vi "DeltaRAWdata(SubVI).vi"(1 "Value 3":u16[][](array[numeric]), 3 "error input":errorcluster) -> (5 "Robot-Delta 2":T1, 8 "error out":errorcluster)   [LabVIEW 2019]
panel:
  in  "Robot-Delta":T1
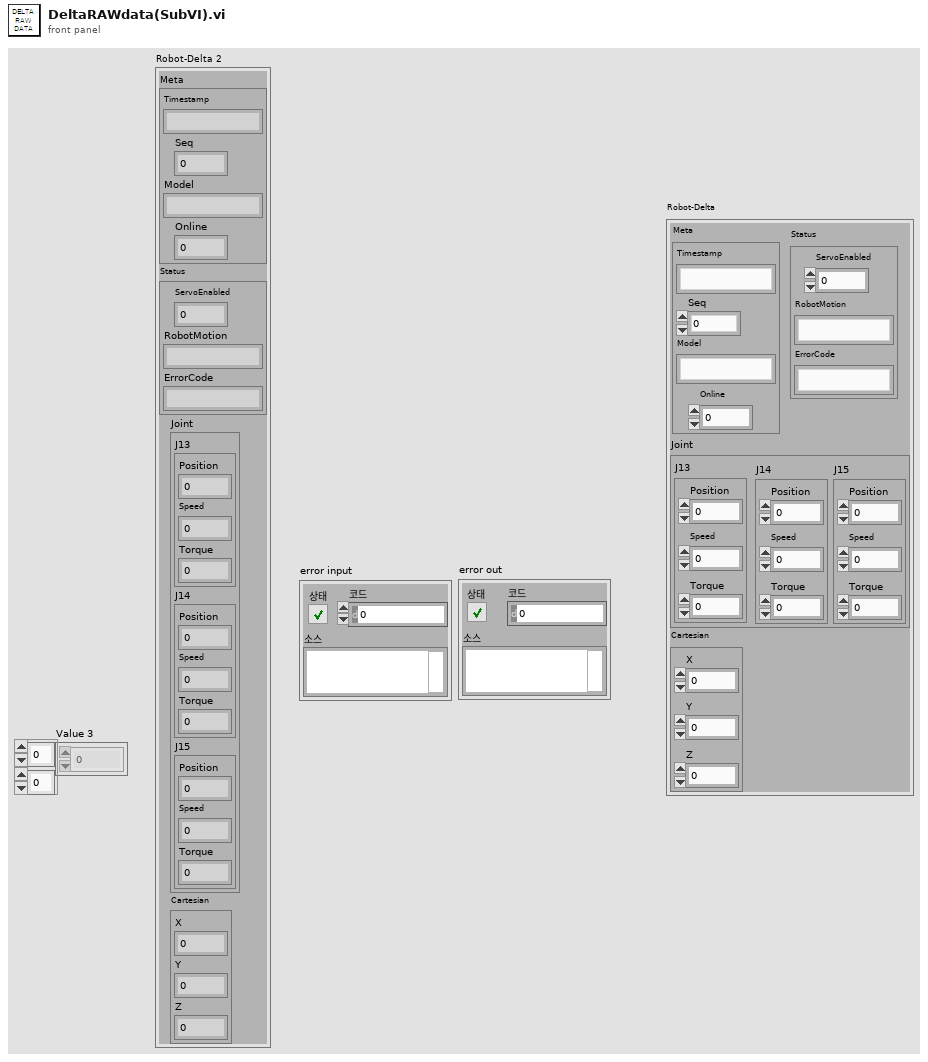
[diagram p1: front panel]
types:
  T1 = cluster{"Meta":cluster{"Timestamp":string, "Seq":dbl, "Model":string, "Online":dbl}, "Status":cluster{"ServoEnabled":dbl, "RobotMotion":string, "ErrorCode":string}, "Joint":cluster{"J13":cluster{"Position":dbl, "Speed":dbl, "Torque":dbl}, "J14":cluster{"Position":dbl, "Speed":dbl, "Torque":dbl}, "J15":cluster{"Position":dbl, "Speed":dbl, "Torque":dbl}}, "Cartesian":cluster{"X":dbl, "Y":dbl, "Z":dbl}}
  T2 = cluster{"[0]":u16, "[1]":u16, "[2]":u16, "[3]":u16, "[4]":u16, "[5]":u16, "[6]":u16, "[7]":u16, "[8]":u16}
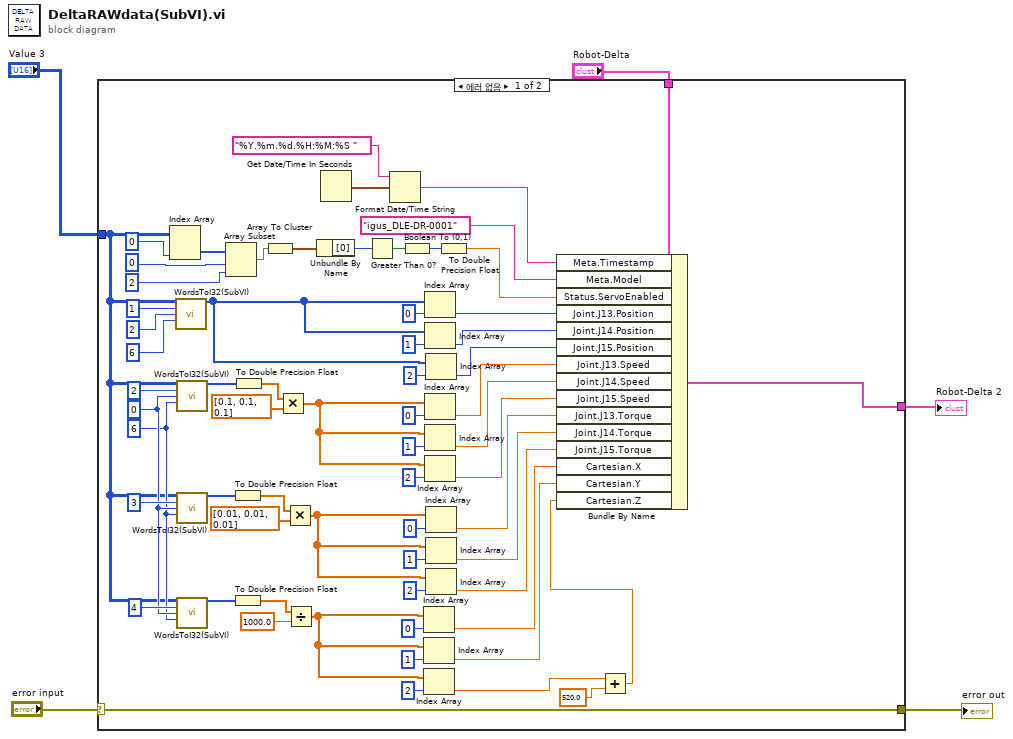
[diagram p0: block diagram]
diagram:
  n1 = case shown="에러 없음" "error input" {
    selector: "error input" -> [w48 w72]
    tunnel: "Value 3" -> [w52 _]
    tunnel: [w48 w72] -> w3
    tunnel: "Robot-Delta" -> [w47 w71]
    tunnel: [w46 w71] -> w1
    frame No Error {
      w57 = 6 ("길이")
      w58 = 0 ("인덱스")
      n2 = Index Array(array=w52, index (col)=0 ("인덱스 (열)")) -> (element=w53:u16[])  [unwired: 1 in]
      n3 = call "WordsToI32(SubVI).vi"("배열"=w52, "인덱스 (열)"=1, "인덱스"=2, "길이"=6) -> ("array output"=w31:i32[])  [unwired: 10 in, 1 out]
      n4 = call "WordsToI32(SubVI).vi"("배열"=w52, "인덱스 (열)"=2, "인덱스"=w58, "길이"=w57) -> ("array output"=w64:i32[])  [unwired: 10 in, 1 out]
      n5 = call "WordsToI32(SubVI).vi"("배열"=w52, "인덱스 (열)"=3, "인덱스"=w58, "길이"=w57) -> ("array output"=w61:i32[])  [unwired: 10 in, 1 out]
      n6 = call "WordsToI32(SubVI).vi"("배열"=w52, "인덱스 (열)"=4, "인덱스"=w58, "길이"=w57) -> ("array output"=w55:i32[])  [unwired: 10 in, 1 out]
      n7 = Array Subset(array=w53, index=0 ("인덱스"), length=2 ("길이")) -> (w18:u16[])
      n8 = To Double Precision Float(number=w61) -> (double precision float=w60:dbl[])
      n9 = To Double Precision Float(number=w55) -> (double precision float=w54:dbl[])
      n10 = To Double Precision Float(number=w64) -> (double precision float=w65:dbl[])
      n11 = Array To Cluster(array=w18) -> (cluster=w17:T2)
      n12 = Multiply(x=w65, y=dbl[] [0.1, 0.1, 0.1]) -> (x*y=w32:dbl[])
      n13 = Multiply(x=w60, y=dbl[] [0.01, 0.01, 0.01]) -> (x*y=w33:dbl[])
      n14 = Divide(x=w54, y=1000.0) -> (x/y=w34:dbl[])
      n15 = Unbundle By Name(w17) -> ("[0]"=w15:u16)
      n16 = Get Date/Time In Seconds() -> (seconds since 1Jan1904=w12:timestamp)
      n17 = Greater Than 0?(x=w15) -> (x > 0?=w14:bool)
      n18 = Format Date/Time String(time format string (%c)="%Y.%m.%d.%H:%M:%S ", seconds (now)=w12) -> (date/time string=w9:string)  [unwired: 1 in]
      n19 = Boolean To (0,1)(Boolean=w14) -> (0, 1=w13:i16)
      n20 = Index Array(array=w34, index=0 ("인덱스")) -> (element=w20:dbl)
      n21 = Index Array(array=w34, index=1 ("인덱스")) -> (element=w19:dbl)
      n22 = Index Array(array=w34, index=2 ("인덱스")) -> (element=w7:dbl)
      n23 = Index Array(array=w31, index=0 ("인덱스")) -> (element=w29:i32)
      n24 = Index Array(array=w31, index=1 ("인덱스")) -> (element=w28:i32)
      n25 = Index Array(array=w32, index=0 ("인덱스")) -> (element=w26:dbl)
      n26 = Index Array(array=w32, index=1 ("인덱스")) -> (element=w25:dbl)
      n27 = Index Array(array=w32, index=2 ("인덱스")) -> (element=w24:dbl)
      n28 = Index Array(array=w31, index=2 ("인덱스")) -> (element=w27:i32)
      n29 = Index Array(array=w33, index=0 ("인덱스")) -> (element=w23:dbl)
      n30 = Index Array(array=w33, index=1 ("인덱스")) -> (element=w22:dbl)
      n31 = Index Array(array=w33, index=2 ("인덱스")) -> (element=w21:dbl)
      n32 = To Double Precision Float(number=w13) -> (double precision float=w16:dbl)
      n33 = Add(x=w7, y=520.0) -> (x+y=w6:dbl)
      n34 = Bundle By Name(cluster=w47, "Meta.Timestamp"=w9, "Meta.Model"="igus_DLE-DR-0001", "Status.ServoEnabled"=w16, "Joint.J13.Position"=w29, "Joint.J14.Position"=w28, "Joint.J15.Position"=w27, "Joint.J13.Speed"=w26, "Joint.J14.Speed"=w25, "Joint.J15.Speed"=w24, "Joint.J13.Torque"=w23, "Joint.J14.Torque"=w22, "Joint.J15.Torque"=w21, "Cartesian.X"=w20, "Cartesian.Y"=w19, "Cartesian.Z"=w6) -> (w46:T1)
    }
    frame Error {
    }
  }
  "error out" <- w3
  "Robot-Delta 2" <- w1
